vi "daqmx watchdog config UI.vi"() -> ()   [LabVIEW 2014, in "DAQmx Watchdog editor node.lvclass"]
doc: "All child modules share this same UI. The UI allows for the configuration of Channels, Parameters, and Error Handling."
uses:
  DAQmx Watchdog editor node.lvclass
  <vilib>/NI/Configuration Framework/Node/NodeRef.ctl
  <vilib>/NI/Configuration Framework/Node/NISE_CEF_Node.lvclass
  <vilib>/NI/AMC/Message Queue.ctl
  <vilib>/NI/AMC/Message.ctl
  <vilib>/NI/Tools/Keyed Array/KeyedArray.ctl
  <vilib>/NI/Configuration Framework/Node/UserEventRef.ctl
  <vilib>/NI/Configuration Framework/Controls/EventCluster.ctl
  <vilib>/NI/DCAF/Tag Editor Core/control module/configuration/error classification setting.ctl
  <vilib>/NI/Tag Bus Module Framework/runtime/error classification.ctl
  <vilib>/NI/Configuration Framework/Node/RefreshUIEvent.ctl
  <vilib>/NI/Configuration Framework/Node/CacheState.ctl
  <vilib>/NI/Configuration Framework/Node/StopEvent.ctl
  <vilib>/NI/Configuration Framework/Node/NodeChangeEvent.ctl
  <vilib>/NI/DCAF/Tag Editor Core/Table API/Available Tag Menu/channel action event.ctl
  <vilib>/NI/DCAF/Tag Editor Core/Table API/Available Tag Menu/dialog output action.ctl
  <vilib>/NI/Tag Bus Module Framework/channel/TBM channel.lvclass
  <vilib>/NI/Tag Bus/tag/tag descriptor.lvclass
  <vilib>/NI/DCAF/Tag Editor Core/Table API/Table Manager/Call Back Ref Type Def.ctl
  <vilib>/NI/DCAF/Tag Editor Core/Configuration Editor/Classes/Engine Parent/Engine Parent Editor Node.lvclass
  <vilib>/NI/DCAF/Tag Editor Core/Configuration Editor/Classes/Module editor node/module editor node.lvclass
  <vilib>/NI/DCAF/Tag Editor Core/Table API/Table Manager/references.ctl
  <vilib>/NI/DCAF/Tag Editor Core/Table API/Table Manager/Menu Definition.ctl
  <vilib>/NI/DCAF/Tag Editor Core/Table API/Table Manager/Menu Options.ctl
  <vilib>/NI/DCAF/Tag Editor Core/Table API/Table Manager/Table Events.ctl
  <vilib>/NI/DCAF/Tag Editor Core/Table API/Table Manager/Menu Select.ctl
  <vilib>/NI/DCAF/Tag Editor Core/control module/editor node/control module editor.lvclass
  module/configuration/DAQmx Watchdog configuration.lvclass
  <vilib>/NI/DCAF/Tag Editor Core/control module/configuration/control module configuration.lvclass/control module configuration.ctl
  <vilib>/NI/Configuration Framework/serializable configuration/NISE_CEF_serializable configuration.lvclass/NISE_CEF_serializable configuration.ctl
  <vilib>/NI/Tag Bus Module Framework/channel/channel classification.ctl
  <vilib>/NI/DCAF/Tag Editor Core/control module/configuration/control module configuration.lvclass
  <vilib>/NI/DCAF/Tag Editor Core/control module/configuration/Write error classifications.vi
  <vilib>/NI/DCAF/Tag Editor Core/control module/editor node/read fixed channel configuration.vi
  <vilib>/NI/DCAF/Tag Editor Core/Configuration Editor/Classes/Module editor node/Read Module Configuration.vi
  <vilib>/Utility/LVClass/Get LV Class Name.vi
  <vilib>/NI/Configuration Framework/error generator/NISE_error generator.vi
  <vilib>/NI/Tag Bus Module Framework/module configuration/TBM module configuration.lvclass
  <vilib>/NI/Configuration Framework/serializable configuration/NISE_CEF_serializable configuration.lvclass
  <vilib>/NI/DCAF/Tag Editor Core/Table API/Listbox/Multi Column Listbox.lvclass
  <vilib>/NI/Configuration Framework/NISE_CEF_TreeControl.lvlib
  <vilib>/NI/DCAF/Tag Editor Core/Table API/Table Manager.lvlib
  <vilib>/NI/DCAF UI Toolkit/Controls/DCAF UI Elements.lvlib
  <vilib>/NI/Tools/Keyed Array/Tools_KeyedArray.lvlib
  <vilib>/NI/AMC/AMC.lvlib
  <vilib>/NI/DCAF/Tag Editor Core/Table API/Table Manager/Table Manager.lvclass
  <vilib>/NI/Tag Bus Module Framework/runtime/TBM module execution interface.lvclass
panel:
  in  "Edge":i32(ring)=10280 items=["Rising"=10280, "Falling"=10171]
  in  "Trigger Source":tag
  in  "Trigger Type":i32(ring)=15996 items=["Digital Edge"=10150, "Time"=15996]
  in  "Enum":i32
  in  "user event out":refnum<user-event>
  in  "Top Level Tab Control":enum32{"Watchdog", "Mapping", "Error Handling"}(tab)
  in  "Trigger on network":bool=TRUE
  in  "Digital States":T1(array[cluster]) caption="Digital Output" {"expiration state" items=["High"=10192, "Low"=10214, "Tristate"=10310, "No Change"=10160]}
  in  "Counter States":T1(array[cluster]) caption="Counter Output" {"expiration state" items=["Low"=10214, "High"=10192, "No Change"=10160]}
  in  "Analog States":T2(array[cluster]) caption="Analog Output" {"output type" items=["Voltage"=10322, "Current"=10134, "No Change"=10160]}
  in  "DAQmx Device Name":tag
  in  "Timeout(s)":dbl=10.0 caption="Watchdog Expiration Timeout (s)" format="%#_13g"
  in  "Channels Listbox":i32(listbox)
  in  "mapall":bool
  in  "mapwriters":bool
  in  "error classifications":T3[](array[typedef])
  in  "node change":T5
  in  "stop event":T6
  in  "cache state":T7
  in  "refresh UI":T8
  in  "user event":T9
  in  "main queue":T10
  in  "node ref":T11
  # "Triggering"
  # "Expiration States"
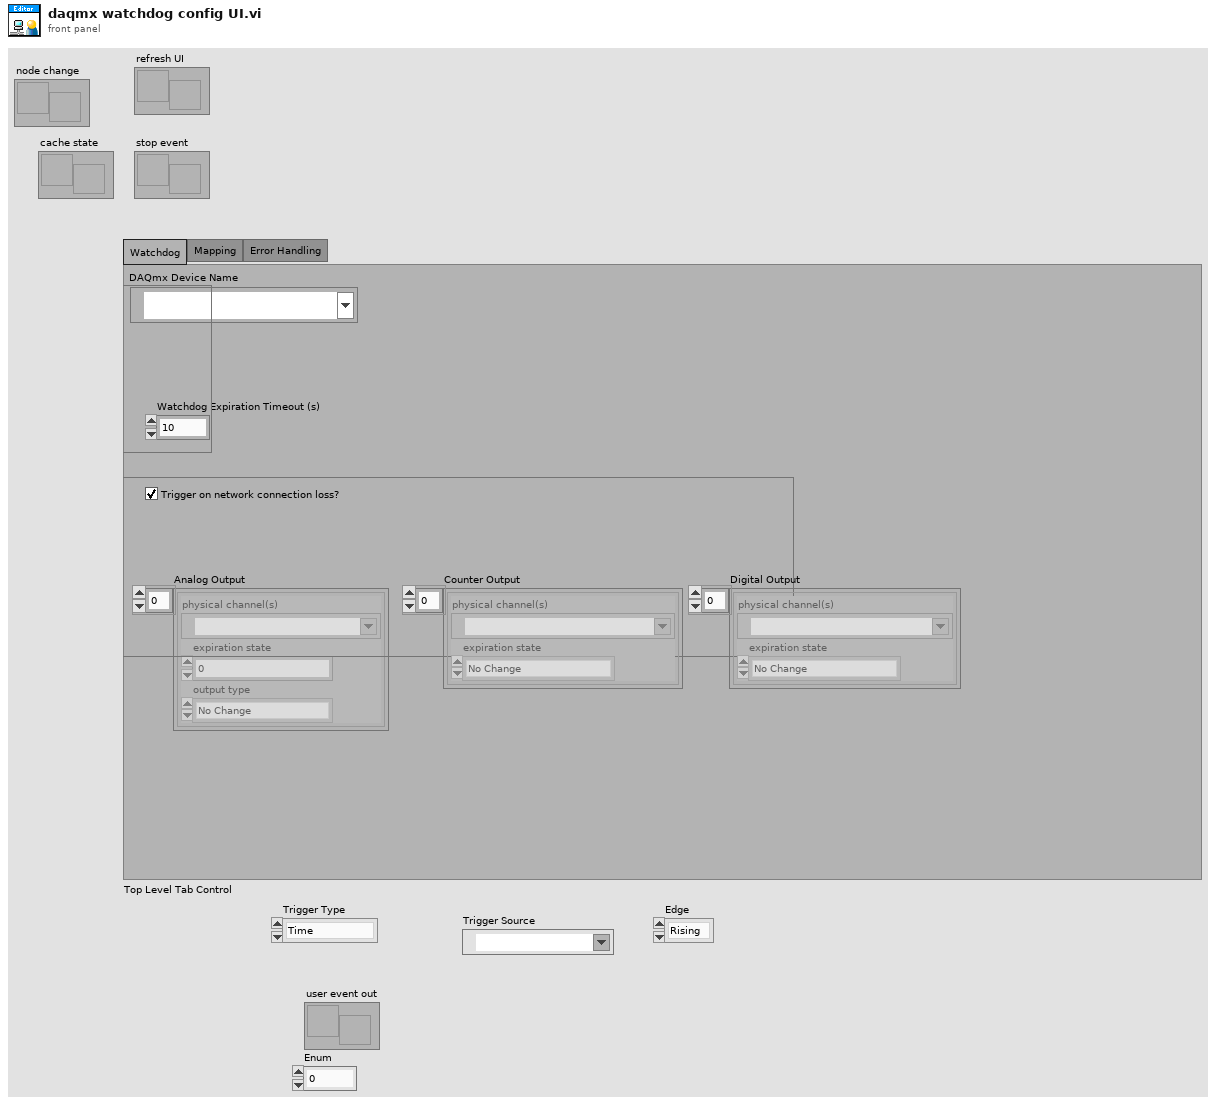
[diagram p1: front panel]
types:
  T1 = cluster{"physical channel(s)":tag, "expiration state":i32}[]
  T2 = cluster{"physical channel":tag, "expiration state":dbl, "output type":i32}[]
  T3 = typedef "control module configuration.lvclass/error classification setting.ctl" = cluster{"code":i32, "error classification":T4}
  T4 = typedef "TBM module execution interface.lvclass/error classification.ctl" = enum16{"unknown", "none", "trivial", "recoverable", "critical"}
  T5 = typedef "NISE_CEF_Node.lvclass/NodeChangeEvent.ctl" = refnum<user-event>
  T6 = typedef "NISE_CEF_Node.lvclass/StopEvent.ctl" = refnum<user-event>
  T7 = typedef "NISE_CEF_Node.lvclass/CacheState.ctl" = refnum<user-event>
  T8 = typedef "NISE_CEF_Node.lvclass/RefreshUIEvent.ctl" = refnum<user-event>
  T9 = typedef "NISE_CEF_Node.lvclass/UserEventRef.ctl" = refnum<user-event>
  T10 = typedef "AMC.lvlib/Message Queue.ctl" = refnum<queue>
  T11 = typedef "NISE_CEF_Node.lvclass/NodeRef.ctl" = refnum<data-value>
  T12 = typedef "Table Manager.lvlib/Table Manager.lvclass/Table Events.ctl" = cluster{"Menu Selection":refnum<user-event>}
  T13 = typedef "Table Manager.lvlib/Table Manager.lvclass/Menu Definition.ctl" = cluster{"Menu Name":string, "Menu Options":T14}
  T14 = typedef "Table Manager.lvlib/Table Manager.lvclass/Menu Options.ctl" = enum16{"Always Show", "Show When Used", "Show When Empty"}
  T15 = typedef "Table Manager.lvlib/Table Manager.lvclass/references.ctl" = cluster{"stop event":T6, "refresh UI":T8, "cache state":T7, "node change":T5, "user event out":refnum<user-event>, "main queue":T10, "user event":T9}
  T16 = typedef "Table Manager.lvlib/Table Manager.lvclass/object ref.ctl" = cluster{"engine":refnum<data-value>, "Node Ref":refnum<data-value>}
  T17 = typedef "Table Manager.lvlib/Column.lvclass/Column Descriptor.ctl" = cluster{"name":string, "caption":string, "Column Type":T18, "Params":string, "AutoSizeMode":i32, "FillWeight":sgl, "MinWidth":u32, "tooltip":string, "Enum Reference":refnum<vi>, "Channel suffix":string, "Read Only":bool, "Call Back VI":T19, "DT Dependency":i32, "name dependency":i32, "data type":T20, "Custom Column":refnum<class "Column.lvclass">}
  T18 = typedef "Table Manager.lvlib/Column.lvclass/Column Type.ctl" = enum16{"String", "Mapping", "Enum", "Custom"}
  T19 = typedef "Table Manager.lvlib/Table Manager.lvclass/Call Back Ref Type Def.ctl" = refnum<vi>
  T20 = typedef "tag bus.lvlib/tag descriptor.lvclass/Data Type.ctl" = enum16{"Double", "Single", "I64", "I32", "I16", "I8", "U64", "U32", "U16", "U8", "Boolean", "String", "Array of Double", "Array of Single", "Array of I64", "Array of I32", "Array of I16", "Array of I8", "Array of U64", "Array of U32", "Array of U16", "Array of U8", "Array of Boolean", "Array of String"}
  T21 = typedef "NISE_CEF_TreeControl.lvlib/EventCluster.ctl" = cluster{"command":string, "data":string}
  T22 = typedef "TBM channel.lvclass/channel classification.ctl" = enum16{"input data", "output data", "processing parameter", "processing result"}
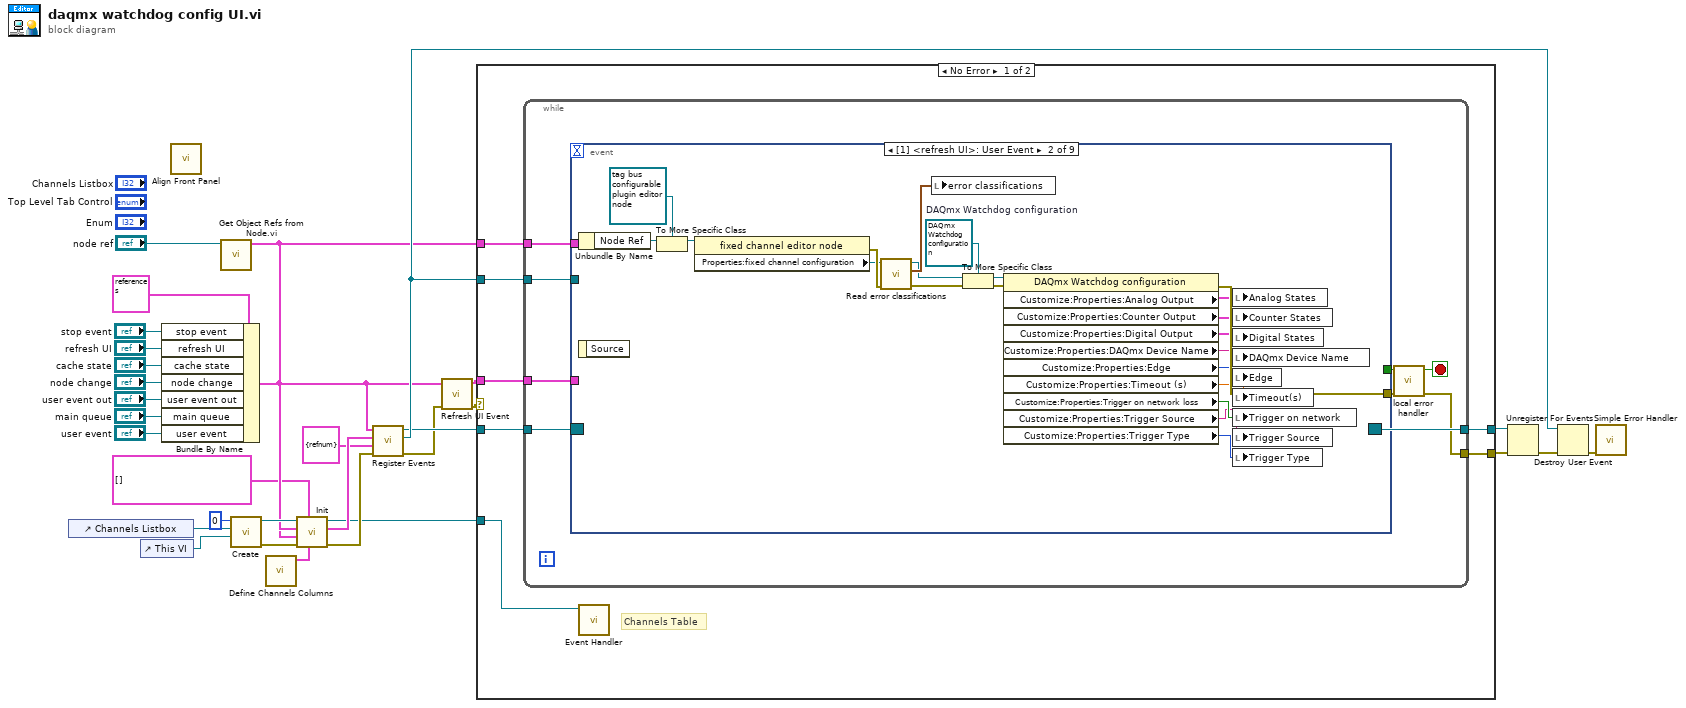
[diagram p0: block diagram]
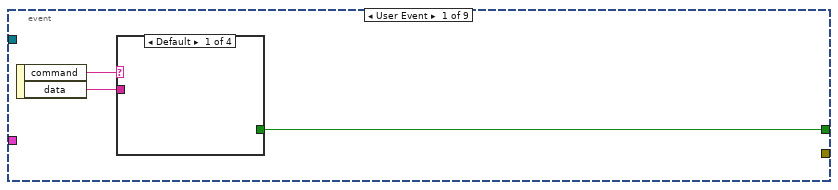
[diagram p2: hidden frame]
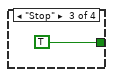
[diagram p4: hidden frame]
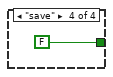
[diagram p5: hidden frame]
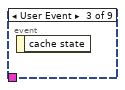
[diagram p6: hidden frame]
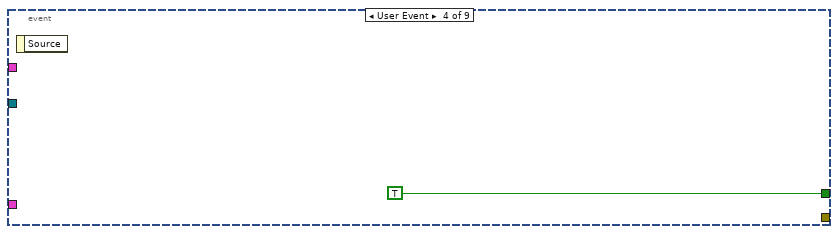
[diagram p7: hidden frame]
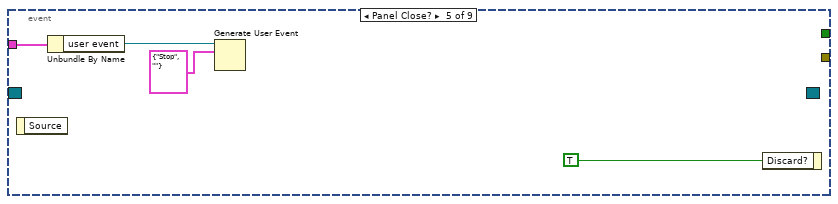
[diagram p8: hidden frame]
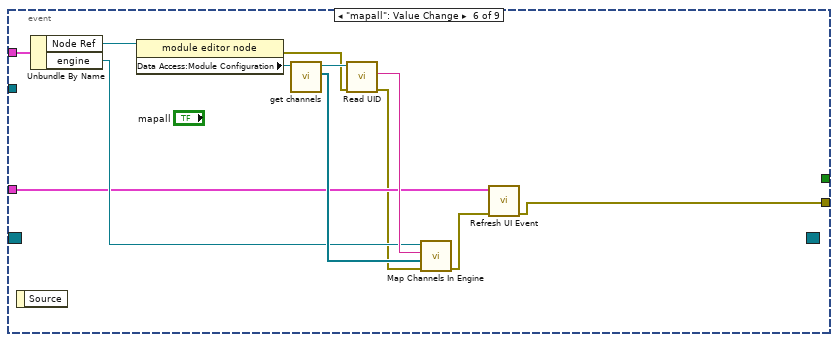
[diagram p9: hidden frame]
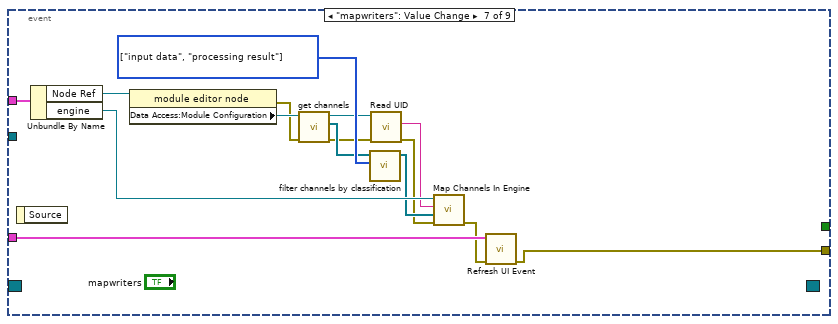
[diagram p10: hidden frame]
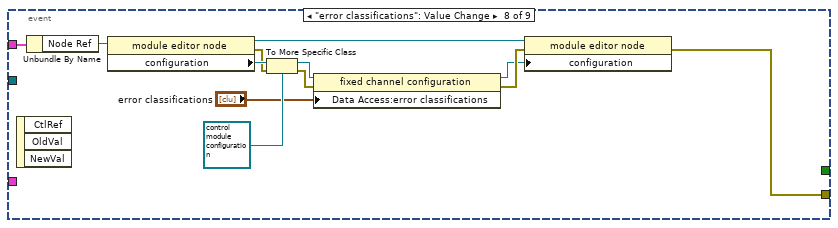
[diagram p11: hidden frame]
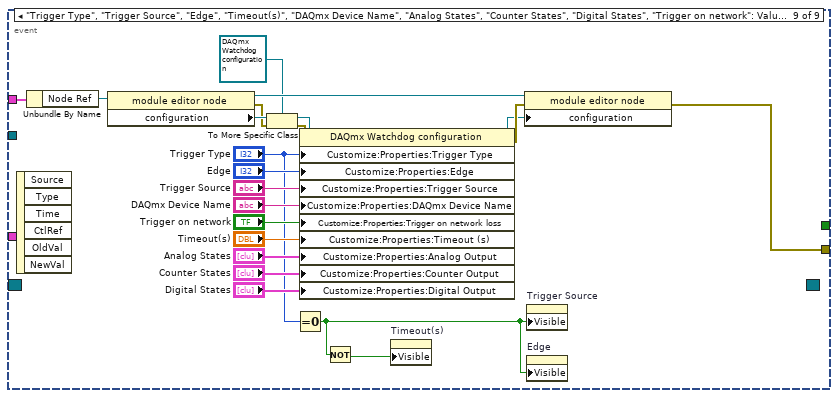
[diagram p12: hidden frame]
diagram:
  n1 = control-ref of="Channels Listbox"() -> (w7:refnum<vi>)
  n2 = control-ref of="This VI"() -> (w6:refnum<vi>)
  n3 = Bundle By Name(cluster=T15 {"stop event"=refnum, "refresh UI"=refnum, "cache state"=refnum, "node change"=refnum, "user event out"=refnum, "main queue"=refnum, "user event"=refnum} ("Event References"), "stop event"="stop event", "refresh UI"="refresh UI", "cache state"="cache state", "node change"="node change", "user event out"="user event out", "main queue"="main queue", "user event"="user event") -> (w5:T15)
  n4 = call <vilib>:"Align Front Panel.vi"() -> ()  [unwired: 10 in, 2 out]
  n5 = call <vilib>:"Get Object Refs from Node.vi.vi"("node ref"="node ref") -> ("Node object refs"=w2:T16)  [unwired: 9 in, 1 out]
  n6 = call <vilib>:"Create.vi"("Top VI"=w6, "Listbox"=w7, "Index"=0) -> ("error out"=w10:errorcluster, "reference out"=w11:refnum<class "Multi Column Listbox.lvclass">)  [unwired: 7 in]
  n7 = call <vilib>:"Define Channels Columns.vi"() -> ("Column Descriptors"=w4:T17[])  [unwired: 11 in]
  n8 = call-dynamic "Init.vi"("Column Descriptors"=w4, "Right-Click Menu"=T13[] [], "error in (no error)"=w10, "Node object refs"=w2, "Event References"=w5, "Multi Column Listbox in"=w11) -> ("error out"=w9:errorcluster, "Table Events"=w21:T12, "Multi Column Listbox out"=w8:refnum<class "Multi Column Listbox.lvclass">)  [unwired: 3 in]
  n9 = call <vilib>:"Register Events.vi"("error in (no error)"=w9, "Parameters Table Events"=T12 {"Menu Selection"=refnum}, "Channels Table Events"=w21, "Event References"=w5) -> ("error out"=w14:errorcluster, "Channel Action"=w20:refnum<user-event>, "Event Registration Refnum"=w19:refnum<event-registration>)  [unwired: 5 in]
  n10 = call <vilib>:"Refresh UI Event.vi"("error in (no error)"=w14, "Event References"=w5) -> ("error out"=w15:errorcluster, "Event References out"=w13:T15)  [unwired: 8 in]
  n11 = case shown="No Error" w15 {
    selector: w15 -> [_ w141]
    tunnel: w19 -> [w38 w140]
    tunnel: [w37 w140] -> w31
    tunnel: [w35 w141] -> w30
    tunnel: w20 -> [w36 _]
    tunnel: w2 -> [w34 _]
    tunnel: w13 -> [w33 _]
    tunnel: w8 -> [w32 _]
    frame No Error {
      # "Channels Table"
      n12 = while {
        tunnel: w38 -> [w47]
        tunnel: [w46] -> w37
        tunnel: w36 -> [w45]
        tunnel: [w41] -> w35
        tunnel: w34 -> [w40]
        tunnel: w33 -> [w39]
        stop <- w43 stop-if-true
        n13 = event shown="[1] <refresh UI>: User Event" {
          selector: w47 -> [_ _ _ _ _ _ _ _ _]
          dyn-events: [_ _ _ _ _ _ _ _ _] -> w46
          timeout: _ -> [_ _ _ _ _ _ _ _ _]
          tunnel: [w50 _ _ TRUE _ _ _ _ _] -> w44
          tunnel: [_ w62 _ _ _ w85 w101 w117 w139] -> w42
          tunnel: w45 -> [_ _ _ _ _ _ _ _ _]
          tunnel: w40 -> [_ w74 _ _ _ w89 w102 w116 w138]
          tunnel: w39 -> [_ _ _ _ w77 w84 w100 _ _]
          event User Event {
            n14 = event-data() -> ("command"=w49:string, "data"=w48:string)  [unwired: 1 in]
            n15 = case shown="Default" w49 {
              tunnel: [_ _ TRUE FALSE] -> w50
              tunnel: w48 -> [_ _ _ _]
              frame Default {
              }
              frame "Refresh" {
              }
              frame "Stop" {
              }
              frame "save" {
              }
            }
          }
          event User Event {
            w65 = refnum<class "DAQmx Watchdog configuration.lvclass"> refnum  # DAQmx Watchdog configuration
            n16 = Unbundle By Name(w74) -> ("Node Ref"=w72:refnum<data-value>)
            n17 = event-data() -> ()  [unwired: 1 in, 1 out]
            n18 = To More Specific Class(target class=refnum<data-value> refnum ("data value reference"), reference=w72) -> (specific class reference=w71:refnum<data-value>)  [unwired: 1 in, 1 out]
            n19 = property class="fixed channel editor node"(reference=w71) -> (error out=w70:errorcluster, "Properties:fixed channel configuration"=w68:refnum<class "control module configuration.lvclass">)  [unwired: 1 in, 1 out]
            n20 = call <vilib>:"Read error classifications.vi"("error in"=w70, "control module configuration in"=w68) -> ("error out"=w66:errorcluster, "error classifications"=w69:T3[], "control module configuration out"=w67:refnum<class "control module configuration.lvclass">)  [unwired: 7 in]
            n21 = local write "error classifications"(w69) -> ()
            n22 = To More Specific Class(target class=w65, reference=w67, error in=w66) -> (specific class reference=w63:refnum<class "DAQmx Watchdog configuration.lvclass">, error out=w64:errorcluster)
            n23 = property class="DAQmx Watchdog configuration"(reference=w63, error in=w64) -> (error out=w62:errorcluster, "Customize:Properties:Analog Output"=w61:T2, "Customize:Properties:Counter Output"=w60:T1, "Customize:Properties:Digital Output"=w59:T1, "Customize:Properties:DAQmx Device Name"=w58:tag, "Customize:Properties:Edge"=w57:i32, "Customize:Properties:Timeout (s)"=w56:dbl, "Customize:Properties:Trigger on network loss"=w55:bool, "Customize:Properties:Trigger Source"=w54:tag, "Customize:Properties:Trigger Type"=w53:i32)  [unwired: 1 out]
            n24 = local write "Analog States"(w61) -> ()
            n25 = local write "Counter States"(w60) -> ()
            n26 = local write "Digital States"(w59) -> ()
            n27 = local write "DAQmx Device Name"(w58) -> ()
            n28 = local write "Edge"(w57) -> ()
            n29 = local write "Timeout(s)"(w56) -> ()
            n30 = local write "Trigger on network"(w55) -> ()
            n31 = local write "Trigger Source"(w54) -> ()
            n32 = local write "Trigger Type"(w53) -> ()
          }
          event User Event {
            n33 = event-data() -> ()  [unwired: 1 in, 1 out]
          }
          event User Event {
            n34 = event-data() -> ()  [unwired: 1 in, 1 out]
          }
          event Panel Close? {
            n35 = event-data() -> ()  [unwired: 1 in, 1 out]
            n36 = Unbundle By Name(w77) -> ("user event"=w76:T9)
            n37 = Generate User Event(user event=w76, event data cluster=T21 {"command"="Stop", "data"=""} ("event data")) -> ()  [unwired: 2 in, 2 out]
            n38 = event-data("Discard?"=TRUE) -> ()  [unwired: 1 in, 1 out]
          }
          event "mapall": Value Change {
            n39 = event-data() -> ()  [unwired: 1 in, 1 out]
            n40 = Unbundle By Name(w89) -> ("Node Ref"=w88:refnum<data-value>, "engine"=w87:refnum<data-value>)
            n41 = property class="module editor node"(reference=w88) -> (error out=w81:errorcluster, "Data Access:Module Configuration"=w83:refnum<class "TBM module configuration.lvclass">)  [unwired: 1 in, 1 out]
            n42 = call-dynamic "get channels.vi"("module configuration in"=w83) -> ("channels"=w91:refnum<class "TBM channel.lvclass">[], "module configuration out"=w82:refnum<class "TBM module configuration.lvclass">)  [unwired: 9 in]
            n43 = call <vilib>:"Read UID.vi"("error in"=w81, "configuration in"=w82) -> ("error out"=w80:errorcluster, "instance id"=w90:string)  [unwired: 7 in, 1 out]
            n44 = call <vilib>:"Map Channels In Engine.vi"("error in (no error)"=w80, "channels"=w91, "instance id"=w90, "Engine DVR"=w87) -> ("error out"=w86:errorcluster)  [unwired: 7 in]
            n45 = call <vilib>:"Refresh UI Event.vi"("error in (no error)"=w86, "Event References"=w84) -> ("error out"=w85:errorcluster)  [unwired: 8 in, 1 out]
          }
          event "mapwriters": Value Change {
            w105 = T22[] [enum."input data", enum."processing result"] items=["input data", "output data", "processing parameter", "processing result"] ("allowed classifications")
            n46 = event-data() -> ()  [unwired: 1 in, 1 out]
            n47 = Unbundle By Name(w102) -> ("Node Ref"=w103:refnum<data-value>, "engine"=w99:refnum<data-value>)
            n48 = property class="module editor node"(reference=w103) -> (error out=w92:errorcluster, "Data Access:Module Configuration"=w94:refnum<class "TBM module configuration.lvclass">)  [unwired: 1 in, 1 out]
            n49 = call-dynamic "get channels.vi"("module configuration in"=w94) -> ("channels"=w104:refnum<class "TBM channel.lvclass">[], "module configuration out"=w93:refnum<class "TBM module configuration.lvclass">)  [unwired: 9 in]
            n50 = call <vilib>:"filter channels by classification.vi"("allowed classifications"=w105, "channels in"=w104) -> ("channels out"=w97:refnum<class "TBM channel.lvclass">[])  [unwired: 9 in]
            n51 = call <vilib>:"Read UID.vi"("error in"=w92, "configuration in"=w93) -> ("error out"=w96:errorcluster, "instance id"=w98:string)  [unwired: 7 in, 1 out]
            n52 = call <vilib>:"Map Channels In Engine.vi"("error in (no error)"=w96, "channels"=w97, "instance id"=w98, "Engine DVR"=w99) -> ("error out"=w95:errorcluster)  [unwired: 7 in]
            n53 = call <vilib>:"Refresh UI Event.vi"("error in (no error)"=w95, "Event References"=w100) -> ("error out"=w101:errorcluster)  [unwired: 8 in, 1 out]
          }
          event "error classifications": Value Change {
            n54 = event-data() -> ()  [unwired: 1 in, 3 out]
            n55 = Unbundle By Name(w116) -> ("Node Ref"=w111:refnum<data-value>)
            n56 = property class="module editor node"(reference=w111) -> (reference out=w115:refnum<data-value>, error out=w107:errorcluster, "configuration"=w110:refnum<class "NISE_CEF_serializable configuration.lvclass">)  [unwired: 1 in]
            n57 = To More Specific Class(target class=refnum<class "control module configuration.lvclass"> refnum ("fixed channel configuration"), reference=w110, error in=w107) -> (specific class reference=w112:refnum<class "control module configuration.lvclass">, error out=w106:errorcluster)
            n58 = property class="fixed channel configuration"(reference=w112, error in=w106, "Data Access:error classifications"="error classifications") -> (reference out=w113:refnum<class "control module configuration.lvclass">, error out=w114:errorcluster)
            n59 = property class="module editor node"(reference=w115, error in=w114, "configuration"=w113) -> (error out=w117:errorcluster)  [unwired: 1 out]
          }
          event "Trigger Type", "Trigger Source", "Edge", "Timeout(s)", "DAQmx Device Name", "Analog States", "Counter States", "Digital States", "Trigger on network": Value Change {
            n60 = event-data() -> ()  [unwired: 1 in, 6 out]
            n61 = Unbundle By Name(w138) -> ("Node Ref"=w133:refnum<data-value>)
            n62 = property class="module editor node"(reference=w133) -> (reference out=w137:refnum<data-value>, error out=w130:errorcluster, "configuration"=w132:refnum<class "NISE_CEF_serializable configuration.lvclass">)  [unwired: 1 in]
            n63 = To More Specific Class(target class=refnum<class "DAQmx Watchdog configuration.lvclass"> refnum ("DAQmx Watchdog configuration"), reference=w132, error in=w130) -> (specific class reference=w134:refnum<class "DAQmx Watchdog configuration.lvclass">, error out=w129:errorcluster)
            n64 = Equal To 0?(x="Trigger Type") -> (x = 0?=w118:bool)
            n65 = property class="DAQmx Watchdog configuration"(reference=w134, error in=w129, "Customize:Properties:Trigger Type"="Trigger Type", "Customize:Properties:Edge"="Edge", "Customize:Properties:Trigger Source"="Trigger Source", "Customize:Properties:DAQmx Device Name"="DAQmx Device Name", "Customize:Properties:Trigger on network loss"="Trigger on network", "Customize:Properties:Timeout (s)"="Timeout(s)", "Customize:Properties:Analog Output"="Analog States", "Customize:Properties:Counter Output"="Counter States", "Customize:Properties:Digital Output"="Digital States") -> (reference out=w135:refnum<class "DAQmx Watchdog configuration.lvclass">, error out=w136:errorcluster)
            n66 = Not(x=w118) -> (.not. x?=w119:bool)
            n67 = property on="Timeout(s)" class="DigNum (strict)"("Visible"=w119) -> ()  [unwired: 2 in, 2 out]
            n68 = property class="module editor node"(reference=w137, error in=w136, "configuration"=w135) -> (error out=w139:errorcluster)  [unwired: 1 out]
            n69 = property on="Trigger Source" class="DAQmxName"("Visible"=w118) -> ()  [unwired: 2 in, 2 out]
            n70 = property on="Edge" class="Ring (strict)"("Visible"=w118) -> ()  [unwired: 2 in, 2 out]
          }
        }
        n71 = call <vilib>:"local error handler.vi"("error in (no error)"=w42, "Stop in"=w44) -> ("error out"=w41:errorcluster, "Stop out"=w43:bool)  [unwired: 8 in]
      }
      n72 = call-dynamic "Event Handler.vi"("Listbox in"=w32) -> ()  [unwired: 9 in, 2 out]
    }
    frame Error {
    }
  }
  n73 = Unregister For Events(event registration refnum=w31, error in=w30) -> (error out=w29:errorcluster)
  n74 = Destroy User Event(user event=w20, error in=w29) -> (error out=w28:errorcluster)
  n75 = call <vilib>:"Simple Error Handler.vi"("error in (no error)"=w28) -> ()  [unwired: 4 in, 5 out]
